vi "Write initialized.vi"(8 "error in (no error)":errorcluster, 10 "initialized":bool, 11 "ZM-HW-hardware in":refnum<class "ZM-HW-hardware.lvclass">) -> (0 "error out":errorcluster, 3 "ZM-HW-hardware out":refnum<class "ZM-HW-hardware.lvclass">)   [LabVIEW 2020, in "ZM-HW-hardware.lvlib" / "ZM-HW-hardware.lvclass"]
doc: "Writes one field of this class's private data. Generated by lvai_create_accessors from the class private data control."
uses:
  ZM-HW-hardware.lvclass
  ZM-HW-hardware.lvclass/ZM-HW-hardware.ctl
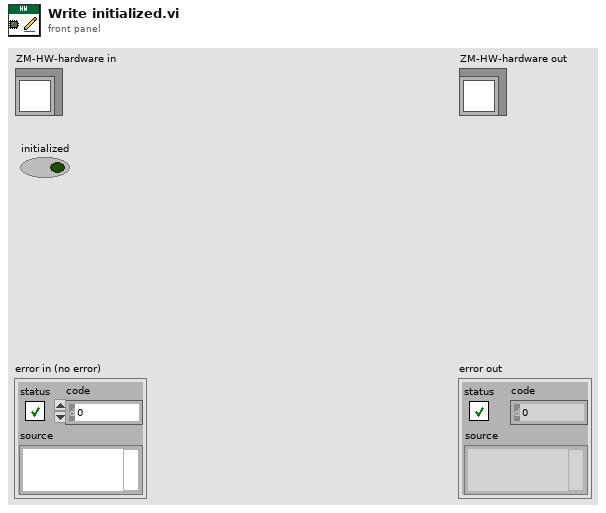
[diagram p1: front panel]
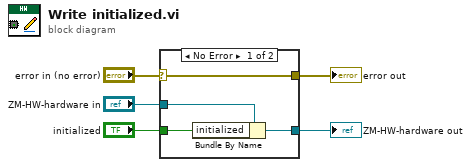
[diagram p0: block diagram]
diagram:
  n1 = case shown="No Error" "error in (no error)" {
    selector: "error in (no error)" -> [w9 w10]
    tunnel: [w9 w10] -> w4
    tunnel: [w7 w11] -> w2
    tunnel: "ZM-HW-hardware in" -> [w8 w11]
    tunnel: "initialized" -> [w6 _]
    frame No Error {
      n2 = Bundle By Name(cluster=w8, "initialized"=w6) -> (w7:refnum<class "ZM-HW-hardware.lvclass">)
    }
    frame Error {
    }
  }
  "error out" <- w4
  "ZM-HW-hardware out" <- w2
